vi "initialize SA Device.vi"(8 "error in (no error)":errorcluster, 9 "S.A Reset?":bool, 10 "VISA resource name":refnum<visa-resource-name>, 11 "FSV-40N in":refnum<class "FSV-40N.lvclass">) -> (0 "error out":errorcluster, 3 "FSV-40N out":refnum<class "FSV-40N.lvclass">)   [LabVIEW 2023, in "Spectrum Analyzer.lvlib" / "FSV-40N.lvclass"]
uses:
  FSV-40N.lvclass
  FSV-40N.lvclass/FSV-40N.ctl
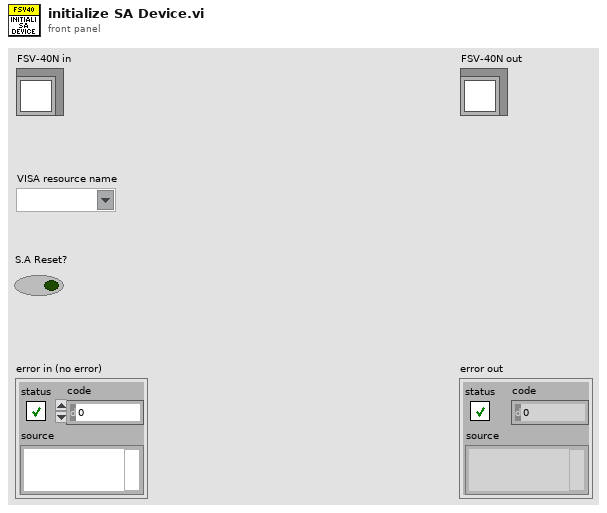
[diagram p1: front panel]
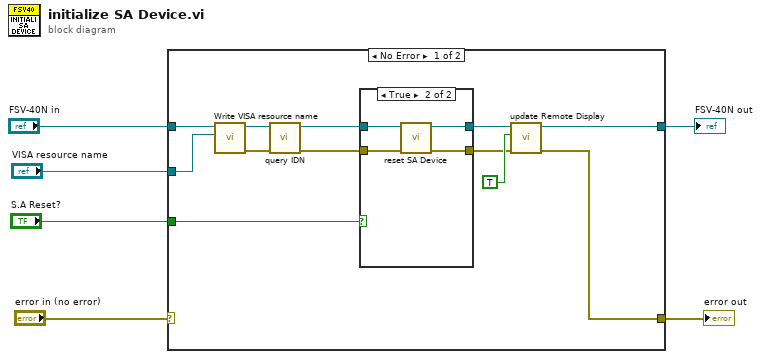
[diagram p0: block diagram]
diagram:
  n1 = case shown="No Error" "error in (no error)" {
    selector: "error in (no error)" -> [_ w26]
    tunnel: "FSV-40N in" -> [w12 w25]
    tunnel: [w15 w26] -> w4
    tunnel: [w18 w25] -> w3
    tunnel: "S.A Reset?" -> [w14 _]
    tunnel: "VISA resource name" -> [w11 _]
    frame No Error {
      n2 = call "Write VISA resource name.vi"("VISA resource name"=w11, "FSV-40N in"=w12) -> ("error out"=w9:errorcluster, "FSV-40N out"=w10:refnum<class "FSV-40N.lvclass">)  [unwired: 8 in]
      n3 = call-dynamic "query IDN.vi"("error in (no error)"=w9, "FSV-40N in"=w10) -> ("error out"=w7:errorcluster, "FSV-40N out"=w8:refnum<class "FSV-40N.lvclass">)  [unwired: 7 in, 1 out]
      n4 = case shown="True" w14 {
        tunnel: w8 -> [w20 w24]
        tunnel: [w20 w23] -> w17
        tunnel: [w19 w22] -> w13
        tunnel: w7 -> [w19 w21]
        frame False {
        }
        frame True {
          n5 = call-dynamic "reset SA Device.vi"("error in (no error)"=w21, "FSV-40N in"=w24) -> ("error out"=w22:errorcluster, "FSV-40N out"=w23:refnum<class "FSV-40N.lvclass">)  [unwired: 8 in]
        }
      }
      n6 = call-dynamic "update Remote Display.vi"("error in (no error)"=w13, "Remote Display On?"=TRUE, "FSV-40N in"=w17) -> ("error out"=w15:errorcluster, "FSV-40N out"=w18:refnum<class "FSV-40N.lvclass">)  [unwired: 7 in]
    }
    frame Error {
    }
  }
  "error out" <- w4
  "FSV-40N out" <- w3
